vi "Ctor.vi"(6 "Name (Caller VI)":string, 8 "error in (no error)":errorcluster) -> (0 "error out":errorcluster, 3 "PanelArray":refnum<class "ArrayManager.lvclass">)   [LabVIEW 2020, in "OOPanel.lvlib" / "ArrayManager.lvclass"]
uses:
  ArrayManager.lvclass
  ArrayPanel/ArrayPanel.lvclass
  UI Refs.ctl
  Events.ctl
  Scroll Into View.ctl
  State Ref.ctl
  Event Regs.ctl
  ArrayManager.lvclass/ArrayManager.ctl
  Manager/Manager.lvclass
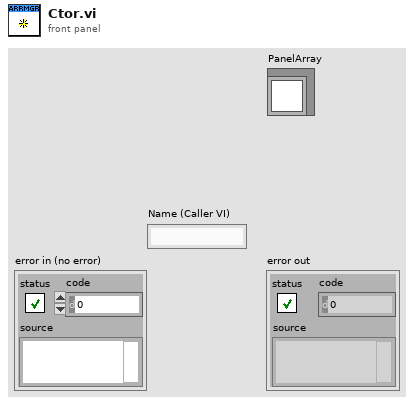
[diagram p1: front panel]
types:
  T1 = typedef "OOPanel.lvlib/ArrayManager.lvclass/Scroll Into View.ctl" = cluster{"Panel Index":i32, "Highlight":bool}
  T2 = typedef "OOPanel.lvlib/ArrayManager.lvclass/Event Regs.ctl" = cluster{"Event Reg":refnum<event-registration>, "Last Update Ticks ms":u32}
  T3 = typedef "OOPanel.lvlib/ArrayManager.lvclass/State Ref.ctl" = cluster{"Running":bool, "Borders":bool, "Total Height":dbl, "Scroll Visible":bool, "Background":u32}
  T4 = typedef "OOPanel.lvlib/ArrayManager.lvclass/Events.ctl" = cluster{"Stop":refnum<user-event>, "Update":refnum<user-event>, "Scroll":refnum<user-event>, "Set BG":refnum<user-event>, "Scroll To Panel":refnum<user-event>, "Highlight":refnum<user-event>}
  T5 = typedef "OOPanel.lvlib/ArrayManager.lvclass/UI Refs.ctl" = cluster{"SubPanels":refnum<vi>[], "Scrollbar":refnum<vi>, "Panel VI":refnum<vi>, "Container":refnum<vi>}
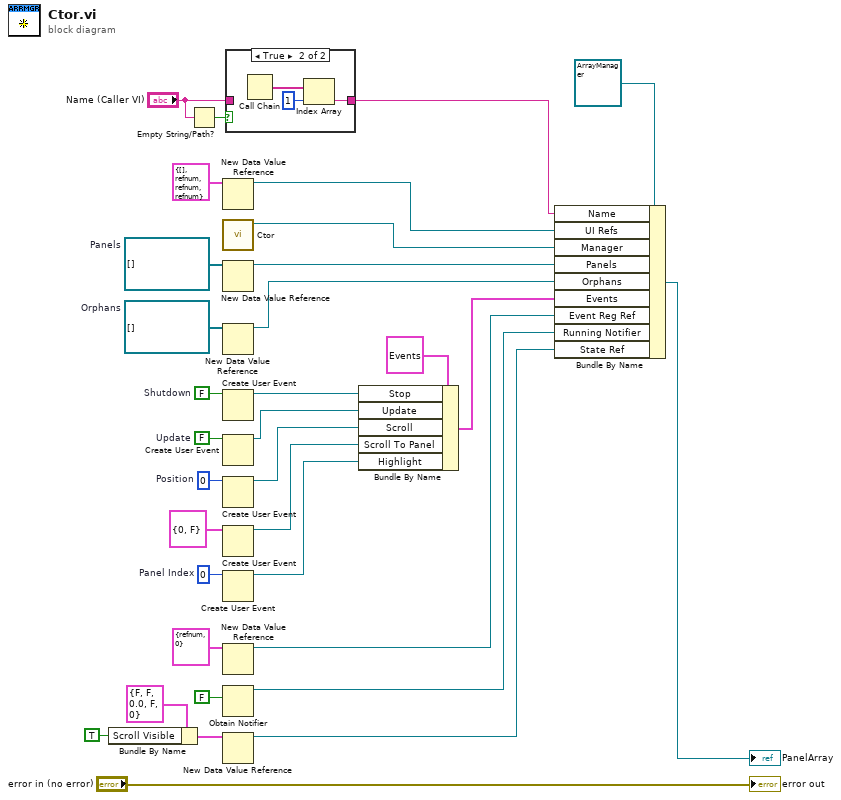
[diagram p0: block diagram]
diagram:
  w2 = 0  # Panel Index
  w12 = 0  # Position
  w20 = FALSE  # Update
  w26 = refnum<class "ArrayPanel.lvclass">[] []  # Orphans
  w27 = refnum<class "ArrayPanel.lvclass">[] []  # Panels
  w29 = FALSE  # Shutdown
  n1 = Bundle By Name(cluster=T3 {"Running"=FALSE, "Borders"=FALSE, "Total Height"=0.0, "Scroll Visible"=FALSE, "Background"=0} ("State Ref"), "Scroll Visible"=TRUE) -> (w14:T3)
  n2 = Empty String/Path?(string/path="Name (Caller VI)") -> (empty?=w7:bool)
  n3 = New Data Value Reference(data value=T5 {"SubPanels"=[], "Scrollbar"=refnum, "Panel VI"=refnum, "Container"=refnum} ("UI Refs")) -> (data value reference=w22:refnum<data-value>)  [unwired: 1 in, 1 out]
  n4 = call "Ctor.vi"() -> ("Manager out"=w30:refnum<class "Manager.lvclass">)  [unwired: 10 in, 1 out]
  n5 = New Data Value Reference(data value=w27) -> (data value reference=w25:refnum<data-value>)  [unwired: 1 in, 1 out]
  n6 = New Data Value Reference(data value=w26) -> (data value reference=w24:refnum<data-value>)  [unwired: 1 in, 1 out]
  n7 = Create User Event(user event datatype=w29) -> (user event=w28:refnum<user-event>)  [unwired: 1 in, 1 out]
  n8 = Create User Event(user event datatype=w20) -> (user event=w19:refnum<user-event>)  [unwired: 1 in, 1 out]
  n9 = Create User Event(user event datatype=w12) -> (user event=w11:refnum<user-event>)  [unwired: 1 in, 1 out]
  n10 = Create User Event(user event datatype=T1 {"Panel Index"=0, "Highlight"=FALSE} ("Scroll Into View")) -> (user event=w3:refnum<user-event>)  [unwired: 1 in, 1 out]
  n11 = Create User Event(user event datatype=w2) -> (user event=w1:refnum<user-event>)  [unwired: 1 in, 1 out]
  n12 = New Data Value Reference(data value=T2 {"Event Reg"=refnum, "Last Update Ticks ms"=0} ("Event Reg State")) -> (data value reference=w8:refnum<data-value>)  [unwired: 1 in, 1 out]
  n13 = Obtain Notifier(notification data type=FALSE) -> (notifier out=w17:refnum<notifier>)  [unwired: 3 in, 2 out]
  n14 = New Data Value Reference(data value=w14) -> (data value reference=w15:refnum<data-value>)  [unwired: 1 in, 1 out]
  n15 = case shown="True" w7 {
    tunnel: "Name (Caller VI)" -> [w34 _]
    tunnel: [w34 w35] -> w5
    frame False {
    }
    frame True {
      n16 = Call Chain() -> (call chain=w37:string[])
      n17 = Index Array(array=w37, index=1) -> (element=w35:string)
    }
  }
  n18 = Bundle By Name(cluster=T4 {"Stop"=refnum, "Update"=refnum, "Scroll"=refnum, "Set BG"=refnum, "Scroll To Panel"=refnum, "Highlight"=refnum} ("Events"), "Stop"=w28, "Update"=w19, "Scroll"=w11, "Scroll To Panel"=w3, "Highlight"=w1) -> (w10:T4)
  n19 = Bundle By Name(cluster=refnum<class "ArrayManager.lvclass"> refnum ("PanelArray in"), "Name"=w5, "UI Refs"=w22, "Manager"=w30, "Panels"=w25, "Orphans"=w24, "Events"=w10, "Event Reg Ref"=w8, "Running Notifier"=w17, "State Ref"=w15) -> (→"PanelArray":refnum<class "ArrayManager.lvclass">)
  "error out" <- "error in (no error)"
